vi "[ex ce]_Array - Index, Subset & Replace.vi"() -> ()   [LabVIEW 2021]
doc: "<B>Example for CalcExpress script syntax</B>\n\nThis VI demonstrates simple methods to read a cell, row, column or subest of 2D array, and replace a subset.\n\n::: CalcExpress Toolkit :::\nCopyright (c) 2000-2026 Konstantin Shifershteyn. All rights reserved."
panel:
  out "Subset":dbl[][](array[numeric])
  out "Cell":dbl
  out "Column":dbl[](array[numeric])
  out "Row":dbl[](array[numeric])
  in  "Expression":string="Cell   = AR1[2,4];            probe(Cell,  \"Cell: scalar\");\nRow    = AR1[1];              probe(Row,   \"Row: 1D array\");\nColumn = AR1[$>,3];           probe(Column,\"Column: 1D array\");\nSubset = AR2[0:1,1:2];        probe(Subset,\"Subset: 2D array\");\nResult = AR1;\nResult[2:$>,1:$>] = Subset;   probe(Result,\"Result: 2D array\");"
  out "Result":dbl[][](array[numeric])
  in  "AR2":dbl[][](array[numeric])=[[-11.0, -12.0, -13.0, -14.0], [-21.0, -22.0, -23.0, -24.0], [-31.0, -32.0, -33.0, -34.0], [-41.0, -42.0, -43.0, -44.0]]
  in  "AR1":dbl[][](array[numeric])=[[11.0, 12.0, 13.0, 14.0, 15.0], [21.0, 22.0, 23.0, 24.0, 25.0], [31.0, 32.0, 33.0, 34.0, 35.0], [41.0, 42.0, 43.0, 44.0, 45.0], [51.0, 52.0, 53.0, 54.0, 55.0]]
  # "Outputs"
  # "Input Arrays"
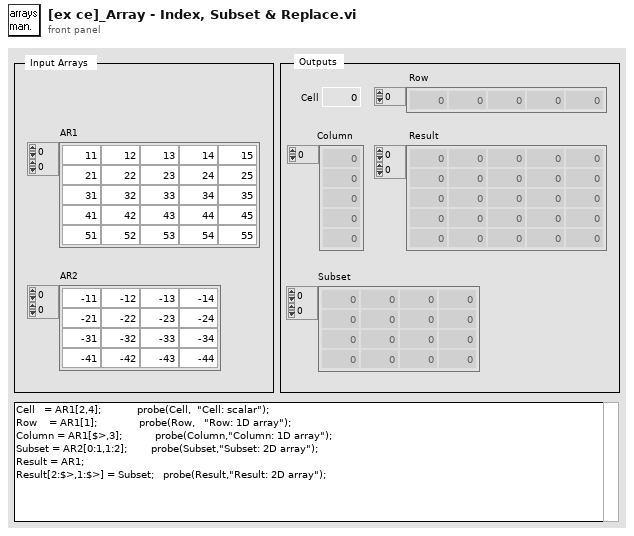
[diagram p1: front panel]
types:
  T1 = enum16{"create", "destroy", "set value", "get value"}
  T2 = typedef "VarMan Variable Context Handle.ctl" = i32
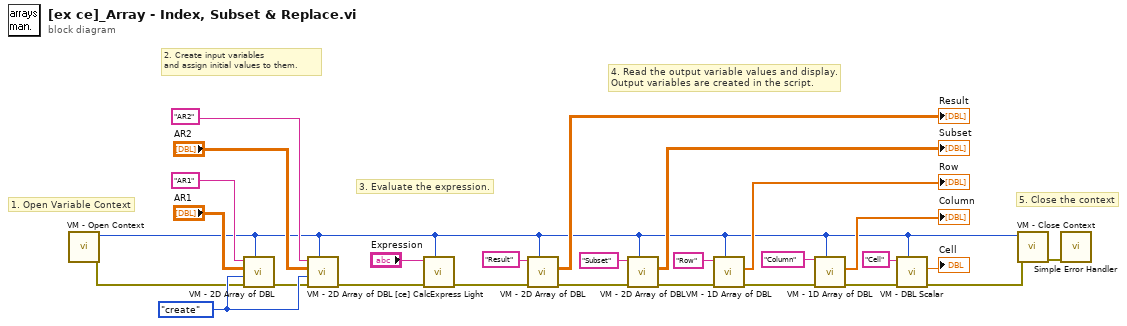
[diagram p0: block diagram]
diagram:
  w15 = T1."create" ("cmd")
  # "5. Close the context"
  # "4. Read the output variable values and display.\nOutput variables are created in the script."
  # "2. Create input variables\nand assign initial values to them."
  # "3. Evaluate the expression."
  # "1. Open Variable Context"
  n1 = call "VM - Open Context.vi"() -> ("error out"=w13:errorcluster, "VC Handle out"=w2:T2)  [unwired: 9 in, 1 out]
  n2 = call "VM - 2D Array of DBL.vi"("VC Handle"=w2, "error in"=w13, "cmd"=w15, "value in"="AR1", "name_spec"="AR1") -> ("error out"=w14:errorcluster)  [unwired: 1 in, 5 out]
  n3 = call "VM - 2D Array of DBL.vi"("VC Handle"=w2, "error in"=w14, "cmd"=w15, "value in"="AR2", "name_spec"="AR2") -> ("error out"=w27:errorcluster)  [unwired: 1 in, 5 out]
  n4 = call "[ce] CalcExpress Light.vi"("VC Handle"=w2, "error in"=w27, "expression"="Expression") -> ("error out"=w8:errorcluster)  [unwired: 6 in, 2 out]
  n5 = call "VM - 2D Array of DBL.vi"("VC Handle"=w2, "error in"=w8, "name_spec"="Result" ("name in")) -> ("error out"=w7:errorcluster, "value out"=→"Result":dbl[][])  [unwired: 3 in, 4 out]
  n6 = call "VM - 2D Array of DBL.vi"("VC Handle"=w2, "error in"=w7, "name_spec"="Subset" ("name in")) -> ("error out"=w6:errorcluster, "value out"=→"Subset":dbl[][])  [unwired: 3 in, 4 out]
  n7 = call "VM - 1D Array of DBL.vi"("VC Handle"=w2, "error in"=w6, "name_spec"="Row" ("name in")) -> ("error out"=w5:errorcluster, "value out"=→"Row":dbl[])  [unwired: 3 in, 4 out]
  n8 = call "VM - 1D Array of DBL.vi"("VC Handle"=w2, "error in"=w5, "name_spec"="Column" ("name in")) -> ("error out"=w4:errorcluster, "value out"=→"Column":dbl[])  [unwired: 3 in, 4 out]
  n9 = call "VM - DBL Scalar.vi"("VC Handle"=w2, "error in"=w4, "name_spec"="Cell" ("name in")) -> ("error out"=w1:errorcluster, "value out"=→"Cell":dbl)  [unwired: 3 in, 4 out]
  n10 = call "VM - Close Context.vi"("error in"=w1, "VC Handle"=w2) -> ("error out"=w3:errorcluster)  [unwired: 8 in, 1 out]
  n11 = call <vilib>:"Simple Error Handler.vi"("error in (no error)"=w3) -> ()  [unwired: 4 in, 5 out]
